vi "Update Numeric Channel Data Types.vi"(8 "error in (no error)":errorcluster, 9 "Size":T1, 11 "Channel in":refnum<class "Channel.lvclass">) -> (0 "error out":errorcluster, 1 "Selected Data Type":T2, 3 "Channel out":refnum<class "Channel.lvclass">)   [LabVIEW 2026, in "Modbus.lvlib" / "Modbus.lvclass"]
uses:
  Modbus.lvclass
  <vilib>/FlexLogger/SDK/PluginSDK.lvlibp/PEFClasses/SDK/Channel/Channel.lvclass
  Types/Numeric Data Type.ctl
  Types/Numeric Size.ctl
  b6b30e35-a115-4b58-8aab-aea09c8000ea.vi
  c3364b71-3b7c-4945-a381-b953504bea10.vi
  c3364b71-3b7c-4945-a381-b953504bea10.vi/407e0540-03f6-4363-afc5-a4b1f046ef19.vi
  c3364b71-3b7c-4945-a381-b953504bea10.vi/520d475a-7b95-4b20-931b-ccc2be82a762.vi
  Globals/Modbus Strings.vi
  <vilib>/FlexLogger/SDK/PluginSDK.lvlibp/PEFClasses/SDK/Channel/ParameterAccess/Read Enum.vi
  <vilib>/FlexLogger/SDK/PluginSDK.lvlibp/PEFClasses/SDK/Channel/ParameterAccess/Write Enum.vi
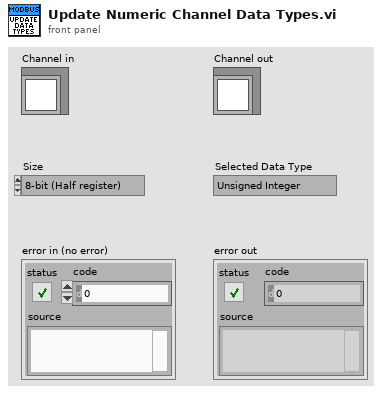
[diagram p1: front panel]
types:
  T1 = typedef "Modbus.lvlib/Modbus.lvclass/Numeric Size.ctl" = enum16{"8-bit (Half register)", "16-bit (One register)", "32-bit (Two registers)", "64-bit (Four registers)"}
  T2 = typedef "Modbus.lvlib/Modbus.lvclass/Numeric Data Type.ctl" = enum16{"Unsigned Integer", "Signed Integer", "Floating Point"}
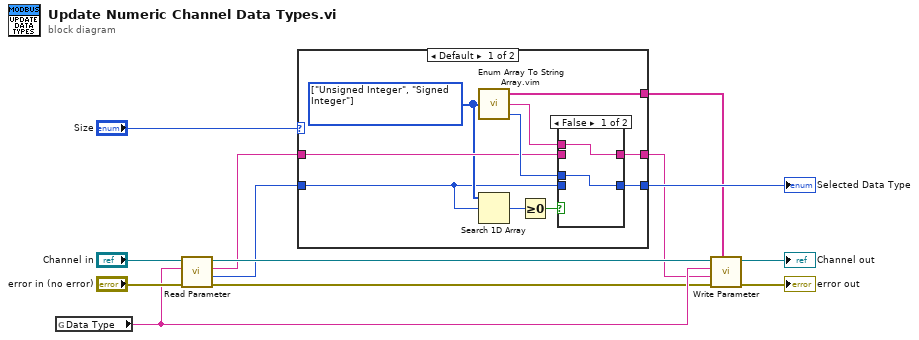
[diagram p0: block diagram]
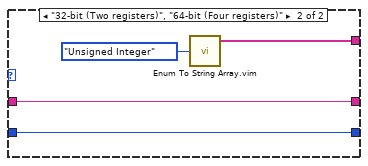
[diagram p3: hidden frame]
diagram:
  n1 = global read "Modbus Strings.vi" "Data Type"() -> (w7:string)
  n2 = call-poly <vilib>:"Read Parameter.vi"("error in (no error)"="error in (no error)", "Name"=w7, "Channel in"="Channel in") -> ("error out"=w5:errorcluster, "Index"=w1:i32, "Value"=w4:string, "Channel out"=w6:refnum<class "Channel.lvclass">)  [unwired: 4 in, 1 out]
  n3 = case shown="Default" "Size" {
    tunnel: [w21 w31] -> w3
    tunnel: [w19 w30] -> w9
    tunnel: w4 -> [w18 w29]
    tunnel: [w20 w29] -> w2
    tunnel: w1 -> [w15 w30]
    frame Default {
      w16 = T2[] [enum."Unsigned Integer", enum."Signed Integer"] items=["Unsigned Integer", "Signed Integer", "Floating Point"]
      n4 = call "Enum Array To String Array.vim"("Array of Enum Values"=w16) -> ("First Value"=w22:T2, "First String"=w23:string, "Strings out"=w21:string[])  [unwired: 2 in]
      n5 = Search 1D Array(1D array=w16, element=w15) -> (index of element=w17:i32)  [unwired: 1 in]
      n6 = Greater Or Equal To 0?(x=w17) -> (x >= 0?=w14:bool)
      n7 = case shown="False" w14 {
        tunnel: w23 -> [w25 _]
        tunnel: w22 -> [w24 _]
        tunnel: [w25 w27] -> w20
        tunnel: [w24 w26] -> w19
        tunnel: w15 -> [_ w26]
        tunnel: w18 -> [_ w27]
        frame False {
        }
        frame True {
        }
      }
    }
    frame "32-bit (Two registers)", "64-bit (Four registers)" {
      n8 = call "Enum To String Array.vim"("Enum in"=Numeric_Data_Type."Unsigned Integer" ("Data Type")) -> ("Strings out"=w31:string[])  [unwired: 2 in, 2 out]
    }
  }
  "Selected Data Type" <- w9
  n9 = call-poly <vilib>:"Write Parameter.vi"("Possible Values"=w3, "error in (no error)"=w5, "Current Value"=w2, "Name"=w7, "Channel in"=w6) -> ("error out"=→"error out":errorcluster, "Channel out"=→"Channel out":refnum<class "Channel.lvclass">)  [unwired: 5 in]
